vi "Untitled 2.vi"() -> ()   [LabVIEW 2021]
panel:
  out "x+y":dbl format="%#_1f"
  in  "stop":bool
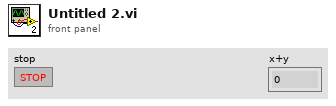
[diagram p1: front panel]
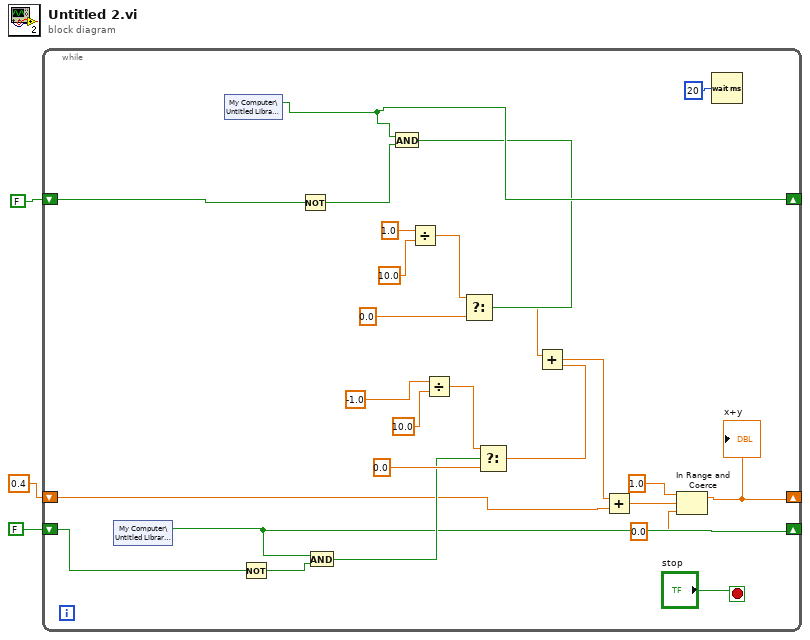
[diagram p0: block diagram]
diagram:
  n1 = while {
    shift-right: [w28] -> _
    shift-left: FALSE -> [w27]
    shift-right: [w8] -> _
    shift-left: FALSE -> [w13]
    shift-right: [w4] -> _
    shift-left: 0.4 ("f") -> [w11]
    stop <- "stop" stop-if-true
    n2 = shared-variable "My Computer\\Untitled Library 2.lvlib\\RT"() -> (w8:bool)  [unwired: 1 in, 1 out]
    n3 = shared-variable "My Computer\\Untitled Library 2.lvlib\\LT"() -> (w28:bool)  [unwired: 1 in, 1 out]
    n4 = Not(x=w13) -> (.not. x?=w18:bool)
    n5 = Not(x=w27) -> (.not. x?=w26:bool)
    n6 = And(x=w8, y=w18) -> (x .and. y?=w12:bool)
    n7 = And(x=w28, y=w26) -> (x .and. y?=w25:bool)
    n8 = Divide(x=1.0, y=10.0) -> (x/y=w24:dbl)
    n9 = Divide(x=-1.0, y=10.0) -> (x/y=w17:dbl)
    n10 = Select(t=w24, s=w25, f=0.0) -> (s? t:f=w19:dbl)
    n11 = Select(t=w17, s=w12, f=0.0) -> (s? t:f=w9:dbl)
    n12 = Add(x=w19, y=w9) -> (x+y=w10:dbl)
    n13 = Add(x=w10, y=w11) -> (x+y=w5:dbl)
    n14 = In Range and Coerce(upper limit=1.0, x=w5, lower limit=0.0) -> (coerced(x)=w4:dbl)  [unwired: 1 out]
    "x+y" <- w4
    n15 = Wait (ms)(milliseconds to wait=u32 20) -> ()  [unwired: 1 out]
  }
